vi "Route FSV Command.vi"(8 "error in (no error)":errorcluster caption="에러 입력(에러 없음)", 10 "문자열":string, 11 "Instrument Manager 입력":refnum<class "Instrument Manager.lvclass">) -> (0 "error out":errorcluster caption="에러 출력", 3 "Instrument Manager 출력":refnum<class "Instrument Manager.lvclass">)   [LabVIEW 2023, in "Instrument Manager.lvclass"]
uses:
  Instrument Manager.lvclass
  <vilib>/regexp/Match Regular Expression.xnode
  Instrument Manager.lvclass/Instrument Manager.ctl
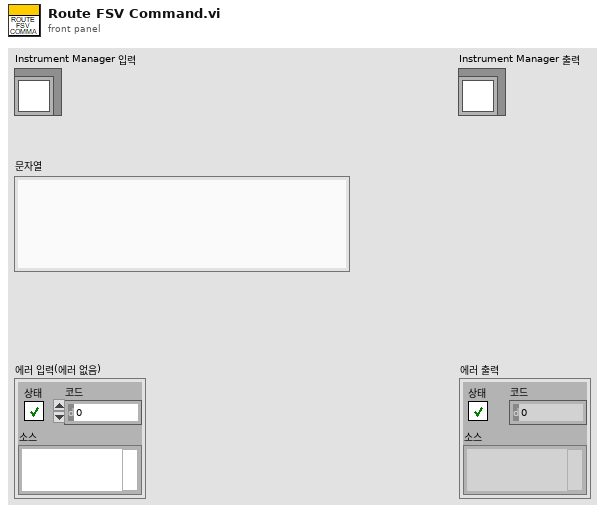
[diagram p1: front panel]
types:
  T1 = typedef "Instrument Manager.lvclass/Connect FSV Params.ctl" = cluster{"type":string, "id":string, "target":string, "command":string, "Params":cluster{"VISA Resource":string}}
  T2 = typedef "Instrument Manager.lvclass/Default Request.ctl" = cluster{"type":string, "id":string, "target":string, "command":string}
  T3 = typedef "Instrument Manager.lvclass/Set TDF File Param.ctl" = cluster{"type":string, "id":string, "target":string, "command":string, "Params":cluster{"TDF File Name":string}}
  T4 = typedef "SA Level Param.ctl" = cluster{"Atten Level":dbl, "Next Peak Search Level":dbl}
  T5 = typedef "Instrument Manager.lvclass/Load SA Level Setting Param.ctl" = cluster{"type":string, "id":string, "target":string, "command":string, "Params":cluster{"SA Level Param":T4}}
  T6 = typedef "SA Range Param.ctl" = cluster{"Start Frequency":dbl, "Stop Frequency":dbl, "RBW":dbl, "VBW":dbl, "Sweep Point":u32, "Limit":dbl}
  T7 = typedef "Instrument Manager.lvclass/Load SA Range Setting Param.ctl" = cluster{"type":string, "id":string, "target":string, "command":string, "Params":cluster{"SA Range Param":T6}}
  T8 = typedef "Instrument Manager.lvclass/Load SA Precision Setting Param.ctl" = cluster{"type":string, "id":string, "target":string, "command":string, "Params":cluster{"Peak Frequency":dbl, "Sweep Time":dbl}}
  T9 = typedef "SA Manual Param.ctl" = cluster{"Start Frequency":dbl, "Stop Frequency":dbl, "RBW":dbl, "VBW":dbl, "Sweep Point":u32, "Sweep Time":dbl, "Atten Level":dbl, "Detector Type":T10, "Limit":dbl}
  T10 = typedef "Spectrum Analyzer.lvlib/TYPE Detect Mode Select.ctl" = enum16{"Det Auto (Normal)", "Auto Peak", "Positive Peak", "Negative Peak", "Sample", "RMS", "Average", "Quasipeak", "CISPR Average", "RMS Average"}
  T11 = typedef "Instrument Manager.lvclass/Load SA Manual Setting Param.ctl" = cluster{"type":string, "id":string, "target":string, "command":string, "Params":cluster{"SA Manual Param":cluster{"Start Frequency":dbl, "Stop Frequency":dbl, "RBW":dbl, "VBW":dbl, "Sweep Point":u32, "Sweep Time":dbl, "Atten Level":dbl, "Detector Mode":string, "Limit":dbl}}}
  T12 = typedef "Instrument Manager.lvclass/Search Fundamental Frequency Param.ctl" = cluster{"type":string, "id":string, "target":string, "command":string, "Params":cluster{"Center Frequency":dbl}}
  T13 = typedef "Spectrum Analyzer.lvlib/TYPE Marker Value.ctl" = cluster{"X-axis":dbl, "Y-axis":dbl}
  T14 = typedef "Instrument Manager.lvclass/Mark Harmonic Param.ctl" = cluster{"type":string, "id":string, "target":string, "command":string, "Params":cluster{"Fundamental Frequency":dbl}}
  T15 = typedef "Instrument Manager.lvclass/Mark InBand Param.ctl" = cluster{"type":string, "id":string, "target":string, "command":string, "Params":cluster{"Limit":dbl}}
  T16 = typedef "Instrument Manager.lvclass/Set Marker Param.ctl" = cluster{"type":string, "id":string, "target":string, "command":string, "Params":cluster{"Marker Index":i32, "Excursion":dbl}}
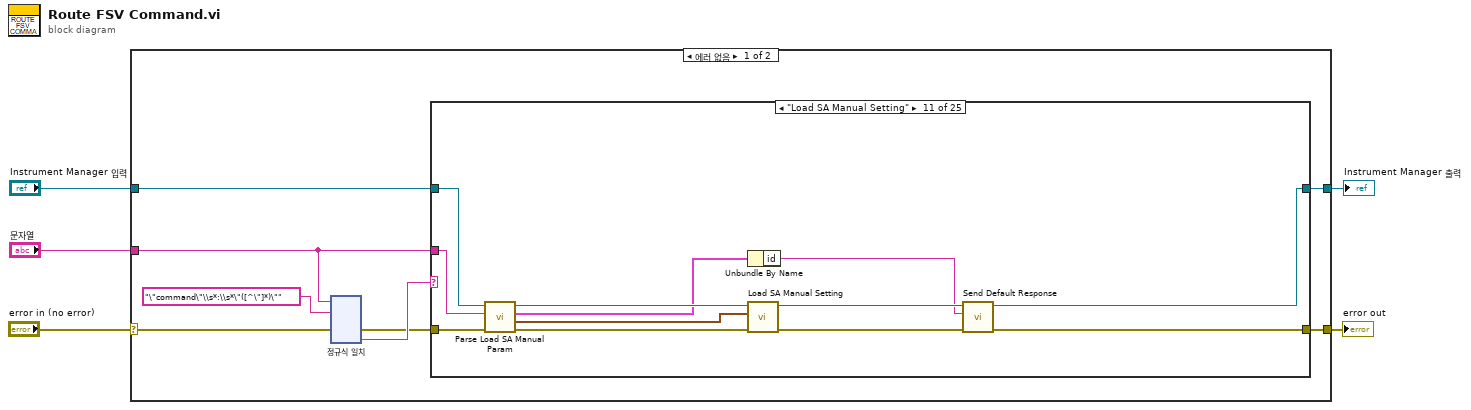
[diagram p0: block diagram]
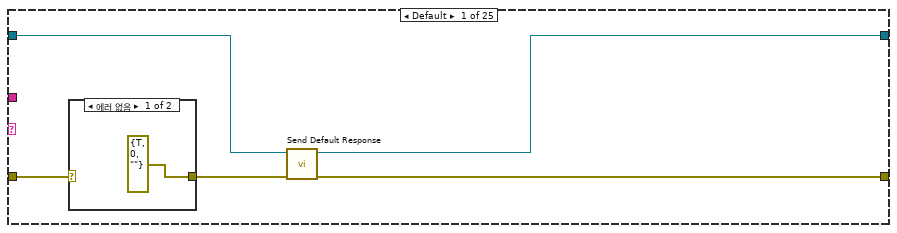
[diagram p2: hidden frame]
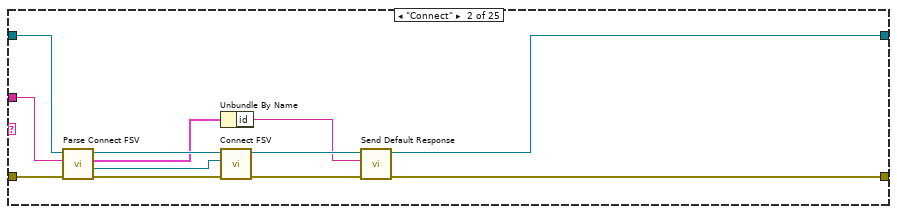
[diagram p4: hidden frame]
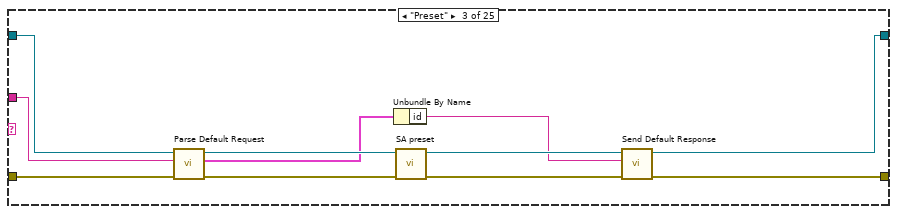
[diagram p5: hidden frame]
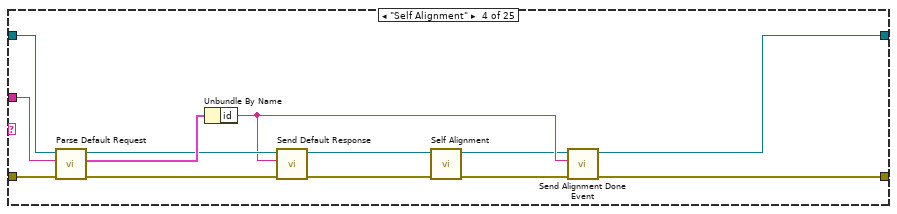
[diagram p6: hidden frame]
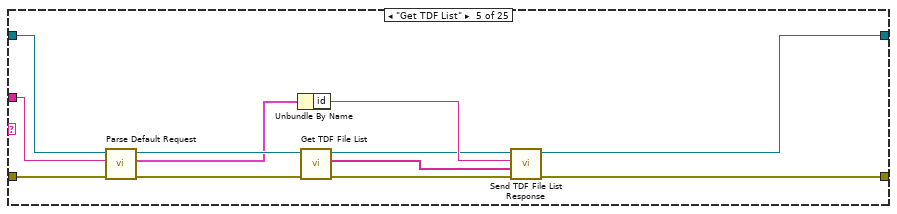
[diagram p7: hidden frame]
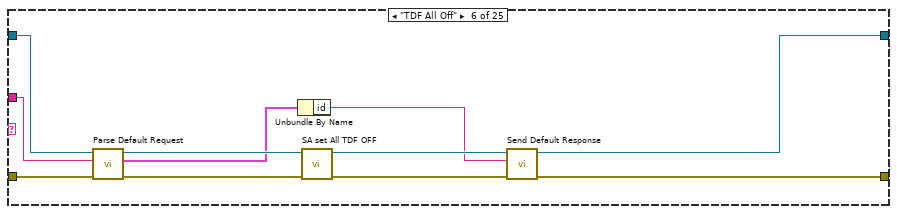
[diagram p8: hidden frame]
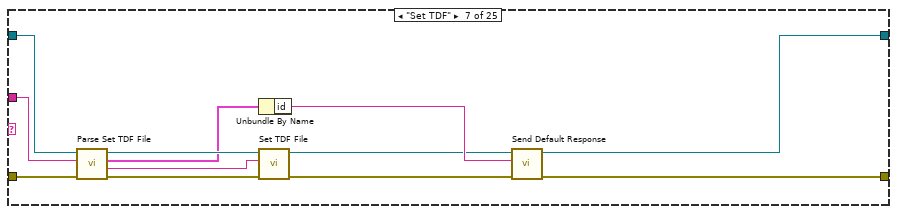
[diagram p9: hidden frame]
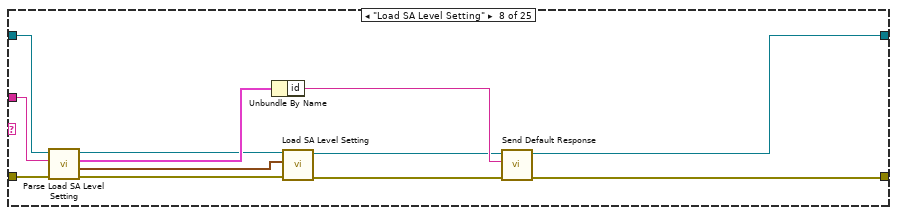
[diagram p10: hidden frame]
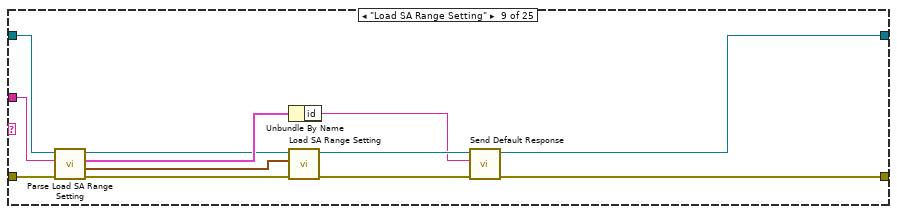
[diagram p11: hidden frame]
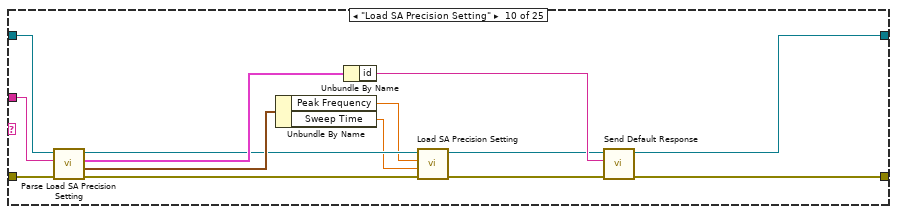
[diagram p12: hidden frame]
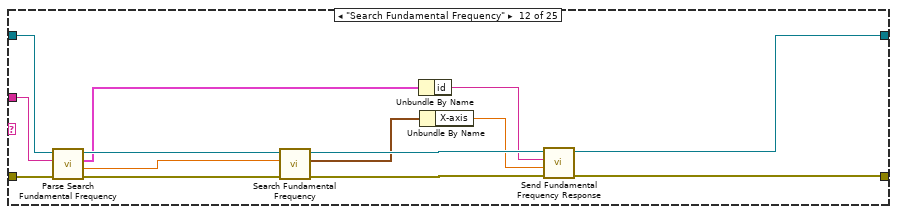
[diagram p13: hidden frame]
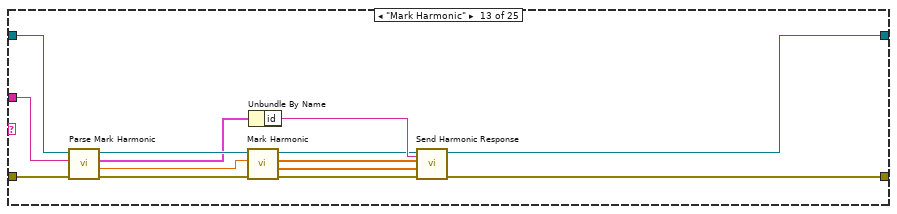
[diagram p14: hidden frame]
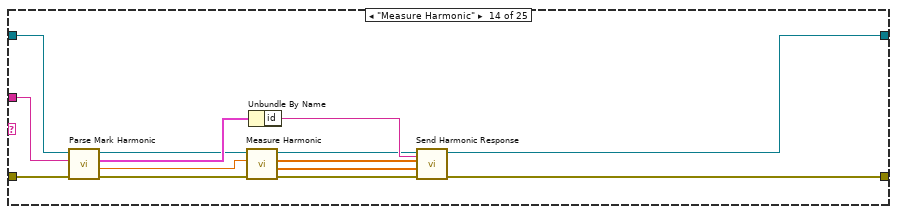
[diagram p15: hidden frame]
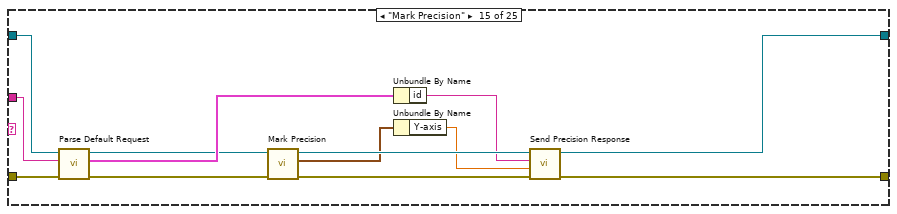
[diagram p16: hidden frame]
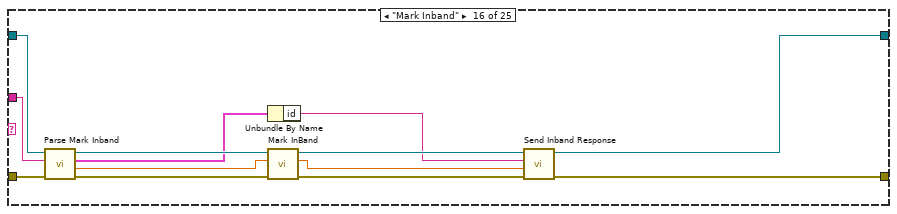
[diagram p17: hidden frame]
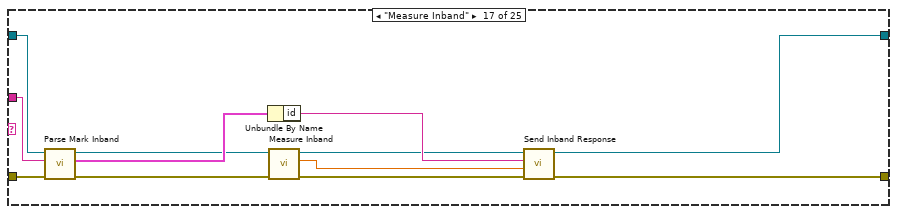
[diagram p18: hidden frame]
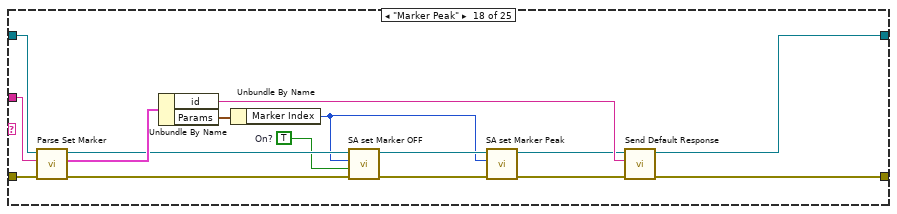
[diagram p19: hidden frame]
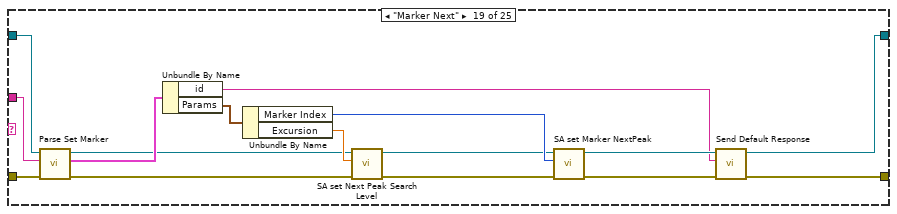
[diagram p20: hidden frame]
diagram:
  n1 = case shown="에러 없음" "error in (no error)" {
    selector: "error in (no error)" -> [w12 w445]
    tunnel: [w9 w445] -> w4
    tunnel: [w6 w444] -> w2
    tunnel: "Instrument Manager 입력" -> [w8 w444]
    tunnel: "문자열" -> [w11 _]
    frame No Error {
      n2 = xnode "정규식 일치"("입력 문자열"=w11, "정규식"="\"command\"\\s*:\\s*\"([^\"]*)\"", "에러 입력"=w12) -> ("에러 출력"=w7:errorcluster, "부분 일치 1"=w10:string)  [unwired: 3 in, 4 out]
      n3 = case shown="\"Load SA Manual Setting\"" w10 {
        tunnel: w11 -> [_ w31 w35 w54 w57 w77 w86 w102 w112 w127 w140 w153 w168 w182 w195 w207 w219 w237 w250 w264 w273 w278 w290 w306 w314]
        tunnel: [w18 w22 w40 w49 w63 w71 w82 w92 w107 w119 w134 w143 w158 w178 w189 w201 w217 w231 w245 w260 w274 w286 w292 w309 w316] -> w9
        tunnel: w8 -> [w15 w32 w36 w55 w67 w78 w87 w101 w111 w128 w139 w154 w169 w183 w196 w208 w220 w235 w249 w265 w272 w285 w293 w308 w315]
        tunnel: w7 -> [w17 w30 w41 w56 w68 w79 w90 w103 w113 w129 w141 w155 w167 w181 w194 w209 w221 w236 w251 w266 w277 w287 w301 w310 w323]
        tunnel: [w14 w21 w39 w48 w58 w74 w81 w93 w104 w116 w130 w142 w157 w177 w188 w200 w216 w226 w239 w254 w267 w282 w291 w302 w313] -> w6
        frame Default {
          n4 = case shown="에러 없음" w17 {
            selector: w17 -> [_ w20]
            tunnel: [errorcluster {"status"=TRUE, "code"=0, "source"=""} ("error IO") w20] -> w16
            frame No Error {
            }
            frame Error {
            }
          }
          n5 = call "Send Default Response.vi"("error in (no error)"=w16, "Instrument Manager 입력"=w15) -> ("error out"=w18:errorcluster, "Instrument Manager 출력"=w14:refnum<class "Instrument Manager.lvclass">)  [unwired: 8 in]
        }
        frame "Connect" {
          n6 = call "Parse Connect FSV.vi"("error in (no error)"=w30, "문자열"=w31, "Instrument Manager 입력"=w32) -> ("error out"=w27:errorcluster, "VISA Resource"=w29:refnum<visa-resource-name>, "Connect FSV Param"=w26:T1, "Instrument Manager 출력"=w28:refnum<class "Instrument Manager.lvclass">)  [unwired: 4 in]
          n7 = Unbundle By Name(w26) -> ("id"=w23:string)
          n8 = call "Connect FSV.vi"("error in (no error)"=w27, "VISA resource name"=w29, "Instrument Manager 입력"=w28) -> ("error out"=w25:errorcluster, "Instrument Manager 출력"=w24:refnum<class "Instrument Manager.lvclass">)  [unwired: 7 in]
          n9 = call "Send Default Response.vi"("error in (no error)"=w25, "id"=w23, "Instrument Manager 입력"=w24) -> ("error out"=w22:errorcluster, "Instrument Manager 출력"=w21:refnum<class "Instrument Manager.lvclass">)  [unwired: 7 in]
        }
        frame "Preset" {
          n10 = call "Parse Default Request.vi"("error in (no error)"=w41, "JSON string"=w35, "Instrument Manager 입력"=w36) -> ("error out"=w42:errorcluster, "Default Request"=w34:T2, "Instrument Manager 출력"=w37:refnum<class "Instrument Manager.lvclass">)  [unwired: 6 in]
          n11 = Unbundle By Name(w34) -> ("id"=w33:string)
          n12 = call "SA preset.vi"("error in (no error)"=w42, "Instrument Manager 입력"=w37) -> ("error out"=w43:errorcluster, "Instrument Manager 출력"=w38:refnum<class "Instrument Manager.lvclass">)  [unwired: 8 in]
          n13 = call "Send Default Response.vi"("error in (no error)"=w43, "id"=w33, "Instrument Manager 입력"=w38) -> ("error out"=w40:errorcluster, "Instrument Manager 출력"=w39:refnum<class "Instrument Manager.lvclass">)  [unwired: 7 in]
        }
        frame "Self Alignment" {
          n14 = call "Parse Default Request.vi"("error in (no error)"=w56, "JSON string"=w54, "Instrument Manager 입력"=w55) -> ("error out"=w52:errorcluster, "Default Request"=w53:T2, "Instrument Manager 출력"=w47:refnum<class "Instrument Manager.lvclass">)  [unwired: 6 in]
          n15 = Unbundle By Name(w53) -> ("id"=w45:string)
          n16 = call "Send Default Response.vi"("error in (no error)"=w52, "id"=w45, "Instrument Manager 입력"=w47) -> ("error out"=w51:errorcluster, "Instrument Manager 출력"=w46:refnum<class "Instrument Manager.lvclass">)  [unwired: 7 in]
          n17 = call "Self Alignment.vi"("error in (no error)"=w51, "Instrument Manager 입력"=w46) -> ("error out"=w50:errorcluster, "Instrument Manager 출력"=w44:refnum<class "Instrument Manager.lvclass">)  [unwired: 8 in]
          n18 = call "Send Alignment Done Event.vi"("error in (no error)"=w50, "id"=w45, "Instrument Manager 입력"=w44) -> ("error out"=w49:errorcluster, "Instrument Manager 출력"=w48:refnum<class "Instrument Manager.lvclass">)  [unwired: 7 in]
        }
        frame "Get TDF List" {
          n19 = call "Parse Default Request.vi"("error in (no error)"=w68, "JSON string"=w57, "Instrument Manager 입력"=w67) -> ("error out"=w66:errorcluster, "Default Request"=w62:T2, "Instrument Manager 출력"=w65:refnum<class "Instrument Manager.lvclass">)  [unwired: 6 in]
          n20 = Unbundle By Name(w62) -> ("id"=w61:string)
          n21 = call "Get TDF File List.vi"("error in (no error)"=w66, "Instrument Manager 입력"=w65) -> ("error out"=w64:errorcluster, "File List"=w60:string[], "Instrument Manager 출력"=w59:refnum<class "Instrument Manager.lvclass">)  [unwired: 7 in]
          n22 = call "Send TDF File List Response.vi"("error in (no error)"=w64, "TDF File List"=w60, "id"=w61, "Instrument Manager 입력"=w59) -> ("error out"=w63:errorcluster, "Instrument Manager 출력"=w58:refnum<class "Instrument Manager.lvclass">)  [unwired: 6 in]
        }
        frame "TDF All Off" {
          n23 = call "Parse Default Request.vi"("error in (no error)"=w79, "JSON string"=w77, "Instrument Manager 입력"=w78) -> ("error out"=w73:errorcluster, "Default Request"=w70:T2, "Instrument Manager 출력"=w76:refnum<class "Instrument Manager.lvclass">)  [unwired: 6 in]
          n24 = Unbundle By Name(w70) -> ("id"=w69:string)
          n25 = call "SA set All TDF OFF.vi"("error in (no error)"=w73, "Instrument Manager 입력"=w76) -> ("error out"=w72:errorcluster, "Instrument Manager 출력"=w75:refnum<class "Instrument Manager.lvclass">)  [unwired: 8 in]
          n26 = call "Send Default Response.vi"("error in (no error)"=w72, "id"=w69, "Instrument Manager 입력"=w75) -> ("error out"=w71:errorcluster, "Instrument Manager 출력"=w74:refnum<class "Instrument Manager.lvclass">)  [unwired: 7 in]
        }
        frame "Set TDF" {
          n27 = call "Parse Set TDF File.vi"("error in (no error)"=w90, "JSON string"=w86, "Instrument Manager 입력"=w87) -> ("error out"=w89:errorcluster, "TDF File Name"=w91:string, "Set TDF File Param"=w85:T3, "Instrument Manager 출력"=w88:refnum<class "Instrument Manager.lvclass">)  [unwired: 5 in]
          n28 = Unbundle By Name(w85) -> ("id"=w84:string)
          n29 = call "Set TDF File.vi"("error in (no error)"=w89, "TDF File Name"=w91, "Instrument Manager 입력"=w88) -> ("error out"=w83:errorcluster, "Instrument Manager 출력"=w80:refnum<class "Instrument Manager.lvclass">)  [unwired: 7 in]
          n30 = call "Send Default Response.vi"("error in (no error)"=w83, "id"=w84, "Instrument Manager 입력"=w80) -> ("error out"=w82:errorcluster, "Instrument Manager 출력"=w81:refnum<class "Instrument Manager.lvclass">)  [unwired: 7 in]
        }
        frame "Load SA Level Setting" {
          n31 = call "Parse Load SA Level Setting.vi"("error in (no error)"=w103, "JSON string"=w102, "Instrument Manager 입력"=w101) -> ("error out"=w99:errorcluster, "SA Level Param"=w100:T4, "Load SA Level Settting Param"=w98:T5, "Instrument Manager 출력"=w97:refnum<class "Instrument Manager.lvclass">)  [unwired: 5 in]
          n32 = Unbundle By Name(w98) -> ("id"=w95:string)
          n33 = call "Load SA Level Setting.vi"("error in (no error)"=w99, "SA Level Param"=w100, "Instrument Manager 입력"=w97) -> ("error out"=w96:errorcluster, "Instrument Manager 출력"=w94:refnum<class "Instrument Manager.lvclass">)  [unwired: 7 in]
          n34 = call "Send Default Response.vi"("error in (no error)"=w96, "id"=w95, "Instrument Manager 입력"=w94) -> ("error out"=w92:errorcluster, "Instrument Manager 출력"=w93:refnum<class "Instrument Manager.lvclass">)  [unwired: 7 in]
        }
        frame "Load SA Range Setting" {
          n35 = call "Parse Load SA Range Setting.vi"("error in (no error)"=w113, "문자열"=w112, "Instrument Manager 입력"=w111) -> ("error out"=w110:errorcluster, "SA Range Param"=w115:T6, "Load SA Range Setting Param"=w114:T7, "Instrument Manager 출력"=w109:refnum<class "Instrument Manager.lvclass">)  [unwired: 5 in]
          n36 = Unbundle By Name(w114) -> ("id"=w105:string)
          n37 = call "Load SA Range Setting.vi"("error in (no error)"=w110, "SA Range Param"=w115, "Instrument Manager 입력"=w109) -> ("error out"=w108:errorcluster, "Instrument Manager 출력"=w106:refnum<class "Instrument Manager.lvclass">)  [unwired: 7 in]
          n38 = call "Send Default Response.vi"("error in (no error)"=w108, "id"=w105, "Instrument Manager 입력"=w106) -> ("error out"=w107:errorcluster, "Instrument Manager 출력"=w104:refnum<class "Instrument Manager.lvclass">)  [unwired: 7 in]
        }
        frame "Load SA Precision Setting" {
          n39 = call "Parse Load SA Precision Setting.vi"("error in (no error)"=w129, "JSON string"=w127, "Instrument Manager 입력"=w128) -> ("error out"=w121:errorcluster, "Params"=w125:cluster{"Peak Frequency":dbl, "Sweep Time":dbl}, "Load SA Precision Setting Param"=w126:T8, "Instrument Manager 출력"=w124:refnum<class "Instrument Manager.lvclass">)  [unwired: 5 in]
          n40 = Unbundle By Name(w125) -> ("Peak Frequency"=w122:dbl, "Sweep Time"=w123:dbl)
          n41 = Unbundle By Name(w126) -> ("id"=w118:string)
          n42 = call "Load SA Precision Setting.vi"("error in (no error)"=w121, "Sweep Time(sec)"=w123, "Center Frequency"=w122, "Instrument Manager 입력"=w124) -> ("error out"=w120:errorcluster, "Instrument Manager 출력"=w117:refnum<class "Instrument Manager.lvclass">)  [unwired: 6 in]
          n43 = call "Send Default Response.vi"("error in (no error)"=w120, "id"=w118, "Instrument Manager 입력"=w117) -> ("error out"=w119:errorcluster, "Instrument Manager 출력"=w116:refnum<class "Instrument Manager.lvclass">)  [unwired: 7 in]
        }
        frame "Load SA Manual Setting" {
          n44 = call "Parse Load SA Manual Param.vi"("error in (no error)"=w141, "JSON string"=w140, "Instrument Manager 입력"=w139) -> ("error out"=w138:errorcluster, "SA Manual Param"=w131:T9, "Load SA Manual Setting Param"=w136:T11, "Instrument Manager 출력"=w137:refnum<class "Instrument Manager.lvclass">)  [unwired: 5 in]
          n45 = Unbundle By Name(w136) -> ("id"=w132:string)
          n46 = call "Load SA Manual Setting.vi"("error in (no error)"=w138, "SA Manual Param"=w131, "Instrument Manager 입력"=w137) -> ("error out"=w135:errorcluster, "Instrument Manager 출력"=w133:refnum<class "Instrument Manager.lvclass">)  [unwired: 7 in]
          n47 = call "Send Default Response.vi"("error in (no error)"=w135, "id"=w132, "Instrument Manager 입력"=w133) -> ("error out"=w134:errorcluster, "Instrument Manager 출력"=w130:refnum<class "Instrument Manager.lvclass">)  [unwired: 7 in]
        }
        frame "Search Fundamental Frequency" {
          n48 = call "Parse Search Fundamental Frequency.vi"("error in (no error)"=w155, "문자열"=w153, "Instrument Manager 입력"=w154) -> ("error out"=w152:errorcluster, "Center Frequency"=w150:dbl, "Search Fundamental Frequency Param"=w149:T12, "Instrument Manager 출력"=w151:refnum<class "Instrument Manager.lvclass">)  [unwired: 5 in]
          n49 = call "Search Fundamental Frequency.vi"("error in (no error)"=w152, "Center Frequency (Hz)"=w150, "Instrument Manager 입력"=w151) -> ("error out"=w148:errorcluster, "Marker Value"=w146:T13, "Instrument Manager 출력"=w147:refnum<class "Instrument Manager.lvclass">)  [unwired: 6 in]
          n50 = Unbundle By Name(w149) -> ("id"=w144:string)
          n51 = Unbundle By Name(w146) -> ("X-axis"=w145:dbl)
          n52 = call "Send Fundamental Frequency Response.vi"("error in (no error)"=w148, "숫자형"=w145, "id"=w144, "Instrument Manager 입력"=w147) -> ("error out"=w143:errorcluster, "Instrument Manager 출력"=w142:refnum<class "Instrument Manager.lvclass">)  [unwired: 6 in]
        }
        frame "Mark Harmonic" {
          n53 = call "Parse Mark Harmonic.vi"("error in (no error)"=w167, "JSON string"=w168, "Instrument Manager 입력"=w169) -> ("error out"=w164:errorcluster, "Fundamental Frequency"=w165:dbl, "Mark Harmonic Param"=w163:T14, "Instrument Manager 출력"=w166:refnum<class "Instrument Manager.lvclass">)  [unwired: 5 in]
          n54 = call "Mark Harmonic.vi"("error in (no error)"=w164, "Fundamental Freq"=w165, "Instrument Manager 입력"=w166) -> ("error out"=w159:errorcluster, "Frequency"=w156:dbl[], "Amplitude"=w160:dbl[], "Instrument Manager 출력"=w161:refnum<class "Instrument Manager.lvclass">)  [unwired: 5 in]
          n55 = Unbundle By Name(w163) -> ("id"=w162:string)
          n56 = call "Send Harmonic Response.vi"("id"=w162, "error in (no error)"=w159, "Frequency"=w156, "Amplitude"=w160, "Instrument Manager 입력"=w161) -> ("error out"=w158:errorcluster, "Instrument Manager 출력"=w157:refnum<class "Instrument Manager.lvclass">)  [unwired: 5 in]
        }
        frame "Measure Harmonic" {
          n57 = call "Parse Mark Harmonic.vi"("error in (no error)"=w181, "JSON string"=w182, "Instrument Manager 입력"=w183) -> ("error out"=w174:errorcluster, "Fundamental Frequency"=w170:dbl, "Mark Harmonic Param"=w180:T14, "Instrument Manager 출력"=w176:refnum<class "Instrument Manager.lvclass">)  [unwired: 5 in]
          n58 = call "Measure Harmonic.vi"("error in (no error)"=w174, "Fundametal Freq"=w170, "Instrument Manager 입력"=w176) -> ("error out"=w173:errorcluster, "Frequency"=w171:dbl[], "Amplitude"=w172:dbl[], "Instrument Manager 출력"=w175:refnum<class "Instrument Manager.lvclass">)  [unwired: 5 in]
          n59 = Unbundle By Name(w180) -> ("id"=w179:string)
          n60 = call "Send Harmonic Response.vi"("id"=w179, "error in (no error)"=w173, "Frequency"=w171, "Amplitude"=w172, "Instrument Manager 입력"=w175) -> ("error out"=w178:errorcluster, "Instrument Manager 출력"=w177:refnum<class "Instrument Manager.lvclass">)  [unwired: 5 in]
        }
        frame "Mark Precision" {
          n61 = call "Parse Default Request.vi"("error in (no error)"=w194, "JSON string"=w195, "Instrument Manager 입력"=w196) -> ("error out"=w192:errorcluster, "Default Request"=w193:T2, "Instrument Manager 출력"=w191:refnum<class "Instrument Manager.lvclass">)  [unwired: 6 in]
          n62 = call "Mark Precision.vi"("error in (no error)"=w192, "Instrument Manager 입력"=w191) -> ("error out"=w190:errorcluster, "Marker Value"=w186:T13, "Instrument Manager 출력"=w187:refnum<class "Instrument Manager.lvclass">)  [unwired: 7 in]
          n63 = Unbundle By Name(w193) -> ("id"=w184:string)
          n64 = Unbundle By Name(w186) -> ("Y-axis"=w185:dbl)
          n65 = call "Send Precision Response.vi"("error in (no error)"=w190, "Amplitude"=w185, "id"=w184, "Instrument Manager 입력"=w187) -> ("error out"=w189:errorcluster, "Instrument Manager 출력"=w188:refnum<class "Instrument Manager.lvclass">)  [unwired: 6 in]
        }
        frame "Mark Inband" {
          n66 = call "Parse Mark Inband.vi"("error in (no error)"=w209, "JSON string"=w207, "Instrument Manager 입력"=w208) -> ("error out"=w204:errorcluster, "Limit"=w205:dbl, "Mark InBand Param"=w203:T15, "Instrument Manager 출력"=w206:refnum<class "Instrument Manager.lvclass">)  [unwired: 5 in]
          n67 = Unbundle By Name(w203) -> ("id"=w198:string)
          n68 = call "Mark InBand.vi"("error in (no error)"=w204, "Limit"=w205, "Instrument Manager 입력"=w206) -> ("error out"=w202:errorcluster, "amplitude"=w197:dbl, "Instrument Manager 출력"=w199:refnum<class "Instrument Manager.lvclass">)  [unwired: 6 in]
          n69 = call "Send Inband Response.vi"("error in (no error)"=w202, "Amplitude"=w197, "id"=w198, "Instrument Manager 입력"=w199) -> ("error out"=w201:errorcluster, "Instrument Manager 출력"=w200:refnum<class "Instrument Manager.lvclass">)  [unwired: 6 in]
        }
        frame "Measure Inband" {
          n70 = call "Parse Mark Inband.vi"("error in (no error)"=w221, "JSON string"=w219, "Instrument Manager 입력"=w220) -> ("error out"=w212:errorcluster, "Mark InBand Param"=w218:T15, "Instrument Manager 출력"=w214:refnum<class "Instrument Manager.lvclass">)  [unwired: 5 in, 1 out]
          n71 = Unbundle By Name(w218) -> ("id"=w215:string)
          n72 = call "Measure Inband.vi"("error in (no error)"=w212, "Instrument Manager 입력"=w214) -> ("error out"=w211:errorcluster, "Y-axis"=w210:dbl, "Instrument Manager 출력"=w213:refnum<class "Instrument Manager.lvclass">)  [unwired: 7 in]
          n73 = call "Send Inband Response.vi"("error in (no error)"=w211, "Amplitude"=w210, "id"=w215, "Instrument Manager 입력"=w213) -> ("error out"=w217:errorcluster, "Instrument Manager 출력"=w216:refnum<class "Instrument Manager.lvclass">)  [unwired: 6 in]
        }
        frame "Marker Peak" {
          w222 = TRUE  # On?
          n74 = call "Parse Set Marker.vi"("error in (no error)"=w236, "JSON string"=w237, "Instrument Manager 입력"=w235) -> ("error out"=w234:errorcluster, "Set Marker Param"=w230:T16, "Instrument Manager 출력"=w228:refnum<class "Instrument Manager.lvclass">)  [unwired: 5 in, 1 out]
          n75 = Unbundle By Name(w230) -> ("id"=w229:string, "Params"=w224:cluster{"Marker Index":i32, "Excursion":dbl})
          n76 = Unbundle By Name(w224) -> ("Marker Index"=w223:i32)
          n77 = call "SA set Marker OFF.vi"("error in (no error)"=w234, "On?"=w222, "Marker Index"=w223, "Instrument Manager 입력"=w228) -> ("error out"=w233:errorcluster, "Instrument Manager 출력"=w227:refnum<class "Instrument Manager.lvclass">)  [unwired: 6 in]
          n78 = call "SA set Marker Peak.vi"("error in (no error)"=w233, "Marker Index"=w223, "Instrument Manager 입력"=w227) -> ("error out"=w232:errorcluster, "Instrument Manager 출력"=w225:refnum<class "Instrument Manager.lvclass">)  [unwired: 7 in]
          n79 = call "Send Default Response.vi"("error in (no error)"=w232, "id"=w229, "Instrument Manager 입력"=w225) -> ("error out"=w231:errorcluster, "Instrument Manager 출력"=w226:refnum<class "Instrument Manager.lvclass">)  [unwired: 7 in]
        }
        frame "Marker Next" {
          n80 = call "Parse Set Marker.vi"("error in (no error)"=w251, "JSON string"=w250, "Instrument Manager 입력"=w249) -> ("error out"=w248:errorcluster, "Set Marker Param"=w253:T16, "Instrument Manager 출력"=w243:refnum<class "Instrument Manager.lvclass">)  [unwired: 5 in, 1 out]
          n81 = Unbundle By Name(w253) -> ("id"=w238:string, "Params"=w252:cluster{"Marker Index":i32, "Excursion":dbl})
          n82 = Unbundle By Name(w252) -> ("Marker Index"=w242:i32, "Excursion"=w244:dbl)
          n83 = call "SA set Next Peak Search Level.vi"("error in (no error)"=w248, "Peak Excursion"=w244, "Instrument Manager 입력"=w243) -> ("error out"=w247:errorcluster, "Instrument Manager 출력"=w241:refnum<class "Instrument Manager.lvclass">)  [unwired: 7 in]
          n84 = call "SA set Marker NextPeak.vi"("error in (no error)"=w247, "Marker Index"=w242, "Instrument Manager 입력"=w241) -> ("error out"=w246:errorcluster, "Instrument Manager 출력"=w240:refnum<class "Instrument Manager.lvclass">)  [unwired: 7 in]
          n85 = call "Send Default Response.vi"("error in (no error)"=w246, "id"=w238, "Instrument Manager 입력"=w240) -> ("error out"=w245:errorcluster, "Instrument Manager 출력"=w239:refnum<class "Instrument Manager.lvclass">)  [unwired: 7 in]
        }
        frame "Marker OFF" {
          n86 = call "Parse Set Marker.vi"("error in (no error)"=w266, "JSON string"=w264, "Instrument Manager 입력"=w265) -> ("error out"=w262:errorcluster, "Marker Index"=w256:i32, "Set Marker Param"=w257:T16, "Instrument Manager 출력"=w259:refnum<class "Instrument Manager.lvclass">)  [unwired: 5 in]
          n87 = Unbundle By Name(w257) -> ("id"=w255:string)
          n88 = call "SA set Marker OFF.vi"("error in (no error)"=w262, "On?"=FALSE, "Marker Index"=w256, "Instrument Manager 입력"=w259) -> ("error out"=w261:errorcluster, "Instrument Manager 출력"=w258:refnum<class "Instrument Manager.lvclass">)  [unwired: 6 in]
          n89 = call "Send Default Response.vi"("error in (no error)"=w261, "id"=w255, "Instrument Manager 입력"=w258) -> ("error out"=w260:errorcluster, "Instrument Manager 출력"=w254:refnum<class "Instrument Manager.lvclass">)  [unwired: 7 in]
        }
        frame "Marker ALL OFF" {
          n90 = call "Parse Default Request.vi"("error in (no error)"=w277, "JSON string"=w273, "Instrument Manager 입력"=w272) -> ("error out"=w276:errorcluster, "Default Request"=w270:T2, "Instrument Manager 출력"=w271:refnum<class "Instrument Manager.lvclass">)  [unwired: 6 in]
          n91 = Unbundle By Name(w270) -> ("id"=w269:string)
          n92 = call "SA set Marker ALL OFF.vi"("error in (no error)"=w276, "Instrument Manager 입력"=w271) -> ("error out"=w275:errorcluster, "Instrument Manager 출력"=w268:refnum<class "Instrument Manager.lvclass">)  [unwired: 8 in]
          n93 = call "Send Default Response.vi"("error in (no error)"=w275, "id"=w269, "Instrument Manager 입력"=w268) -> ("error out"=w274:errorcluster, "Instrument Manager 출력"=w267:refnum<class "Instrument Manager.lvclass">)  [unwired: 7 in]
        }
        frame "Marker Auto MAX" {
          n94 = call "Parse Set Marker.vi"("error in (no error)"=w287, "JSON string"=w278, "Instrument Manager 입력"=w285) -> ("error out"=w289:errorcluster, "Marker Index"=w279:i32, "Set Marker Param"=w281:T16, "Instrument Manager 출력"=w284:refnum<class "Instrument Manager.lvclass">)  [unwired: 5 in]
          n95 = Unbundle By Name(w281) -> ("id"=w280:string)
          n96 = call "SA set Marker Auto MAX.vi"("error in (no error)"=w289, "Marker Index"=w279, "Instrument Manager 입력"=w284) -> ("error out"=w288:errorcluster, "Instrument Manager 출력"=w283:refnum<class "Instrument Manager.lvclass">)  [unwired: 7 in]
          n97 = call "Send Default Response.vi"("error in (no error)"=w288, "id"=w280, "Instrument Manager 입력"=w283) -> ("error out"=w286:errorcluster, "Instrument Manager 출력"=w282:refnum<class "Instrument Manager.lvclass">)  [unwired: 7 in]
        }
        frame "Marker set Center" {
          n98 = call "Parse Set Marker.vi"("error in (no error)"=w301, "JSON string"=w290, "Instrument Manager 입력"=w293) -> ("error out"=w300:errorcluster, "Marker Index"=w295:i32, "Set Marker Param"=w298:T16, "Instrument Manager 출력"=w296:refnum<class "Instrument Manager.lvclass">)  [unwired: 5 in]
          n99 = Unbundle By Name(w298) -> ("id"=w297:string)
          n100 = call "SA set Marker Center.vi"("error in (no error)"=w300, "Marker Index"=w295, "Instrument Manager 입력"=w296) -> ("error out"=w299:errorcluster, "Instrument Manager 출력"=w294:refnum<class "Instrument Manager.lvclass">)  [unwired: 7 in]
          n101 = call "Send Default Response.vi"("error in (no error)"=w299, "id"=w297, "Instrument Manager 입력"=w294) -> ("error out"=w292:errorcluster, "Instrument Manager 출력"=w291:refnum<class "Instrument Manager.lvclass">)  [unwired: 7 in]
        }
        frame "Clear Trace" {
          n102 = call "Parse Default Request.vi"("error in (no error)"=w310, "JSON string"=w306, "Instrument Manager 입력"=w308) -> ("error out"=w312:errorcluster, "Default Request"=w305:T2, "Instrument Manager 출력"=w307:refnum<class "Instrument Manager.lvclass">)  [unwired: 6 in]
          n103 = Unbundle By Name(w305) -> ("id"=w304:string)
          n104 = call "Clear Trace.vi"("error in (no error)"=w312, "Instrument Manager 입력"=w307) -> ("error out"=w311:errorcluster, "Instrument Manager 출력"=w303:refnum<class "Instrument Manager.lvclass">)  [unwired: 8 in]
          n105 = call "Send Default Response.vi"("error in (no error)"=w311, "id"=w304, "Instrument Manager 입력"=w303) -> ("error out"=w309:errorcluster, "Instrument Manager 출력"=w302:refnum<class "Instrument Manager.lvclass">)  [unwired: 7 in]
        }
        frame "Get Screenshot" {
          n106 = call "Parse Default Request.vi"("error in (no error)"=w323, "JSON string"=w314, "Instrument Manager 입력"=w315) -> ("error out"=w322:errorcluster, "Default Request"=w318:T2, "Instrument Manager 출력"=w320:refnum<class "Instrument Manager.lvclass">)  [unwired: 6 in]
          n107 = Unbundle By Name(w318) -> ("id"=w317:string)
          n108 = call "SA save Screenshot.vi"("error in (no error)"=w322, "File Name"="screenshot.png", "Instrument Manager 입력"=w320) -> ("error out"=w321:errorcluster, "Instrument Manager 출력"=w319:refnum<class "Instrument Manager.lvclass">)  [unwired: 7 in]
          n109 = call "Send Default Response.vi"("error in (no error)"=w321, "id"=w317, "Instrument Manager 입력"=w319) -> ("error out"=w316:errorcluster, "Instrument Manager 출력"=w313:refnum<class "Instrument Manager.lvclass">)  [unwired: 7 in]
        }
      }
    }
    frame Error {
    }
  }
  "error out" <- w4
  "Instrument Manager 출력" <- w2
